vi "Suppression_segment EPC.vi"(0 "Programme_entrée":cluster{"chaîne":string, "Valeur":dbl}[][](array[cluster]), 1 "Numéro du segment à supprimer":u8) -> (2 "Programme_sortie":cluster{"chaîne":string, "Valeur":dbl}[][](array[cluster]))   [LabVIEW 2022 SP3]
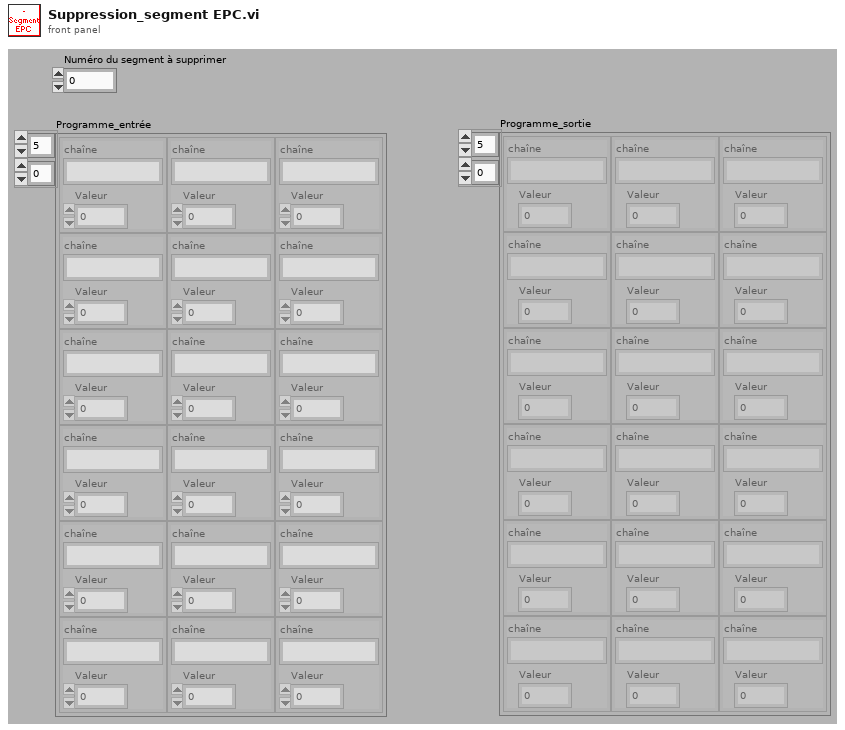
[diagram p1: front panel]
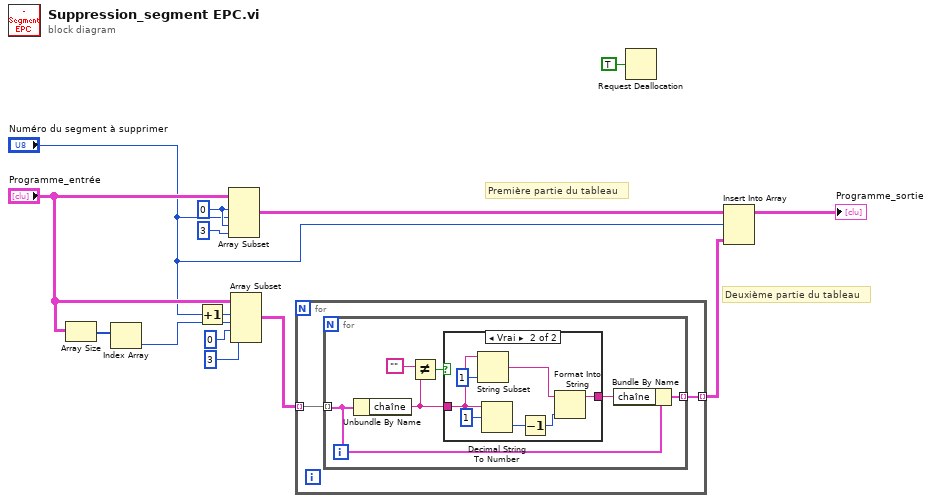
[diagram p0: block diagram]
diagram:
  w10 = 0 ("indice")
  # "Deuxième partie du tableau"
  # "Première partie du tableau"
  n1 = Array Size(array="Programme_entrée") -> (size(s)=w12:i32[])
  n2 = Index Array(array=w12) -> (element=w11:i32)  [unwired: 1 in]
  n3 = Increment(x="Numéro du segment à supprimer") -> (x+1=w14:u8)
  n4 = Array Subset(array="Programme_entrée", index (row)=w10, length (row)="Numéro du segment à supprimer", index (col)=w10, length (col)=3 ("longueur")) -> (w6:cluster{"chaîne":string, "Valeur":dbl}[][])
  n5 = Array Subset(array="Programme_entrée", index (row)=w14, length (row)=w11, index (col)=0 ("indice"), length (col)=3 ("longueur")) -> (w2:cluster{"chaîne":string, "Valeur":dbl}[][])
  n6 = for {
    tunnel: w2 -> [w16] mode=indexing
    tunnel: [w15] -> w1 mode=indexing
    n7 = for {
      tunnel: w16 -> [w22] mode=indexing
      tunnel: [w20] -> w15 mode=indexing
      n8 = Unbundle By Name(w22) -> ("chaîne"=w19:string)
      n9 = Not Equal?(x="", y=w19) -> (x != y?=w17:bool)
      n10 = case shown="Vrai" w17 {
        tunnel: [w23 w25] -> w21
        tunnel: w19 -> [w23 w24]
        frame False {
        }
        frame True {
          n11 = String Subset(string=w24, length (rest)=1 ("longueur (reste)")) -> (substring=w26:string)  [unwired: 1 in]
          n12 = Decimal String To Number(string=w24, offset=1) -> (number=w30:i32)  [unwired: 1 in, 1 out]
          n13 = Decrement(x=w30) -> (x-1=w29:i32)
          n14 = Format Into String(initial string=w26, w29) -> (resulting string=w25:string)  [unwired: 2 in, 1 out]
        }
      }
      n15 = Bundle By Name(cluster=w22, "chaîne"=w21) -> (w20:cluster{"chaîne":string, "Valeur":dbl})
    }
  }
  n16 = Request Deallocation(TRUE ("flag")) -> ()
  n17 = Insert Into Array(array=w6, index (row)="Numéro du segment à supprimer", new element=w1) -> (→"Programme_sortie":cluster{"chaîne":string, "Valeur":dbl}[][])  [unwired: 1 in]
